vi "Create Accounts Fixture.vi"(8 "error in":errorcluster, 11 "Fixture Name":string) -> (0 "error out":errorcluster, 3 "Accounts File Path":path)   [LabVIEW 2026]
doc: "Test support for the ATM Caraya tests. Writes a fresh accounts file with the four records of the exam specification (12345 John Doe 550, 23456 Jennifer Rodriguez 1000, 34567 Bryan Smith 750, 45678 Julie Ramirez 900) to Tests\\results\\<Fixture Name>.txt and returns its path. The results folder is located relative to this VI (one folder up from Support) and created when missing, so the tests run from any checkout location. An existing fixture file is replaced, so every test starts from the same state. Give every test case its own Fixture Name: Caraya runs the cases of one test VI in parallel."
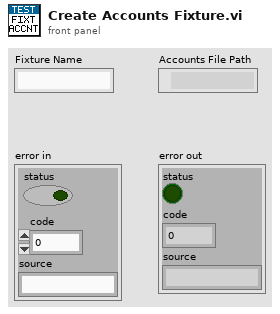
[diagram p1: front panel]
types:
  T1 = enum16{"open", "replace", "create", "open or create", "replace or create", "replace or create with confirmation"}
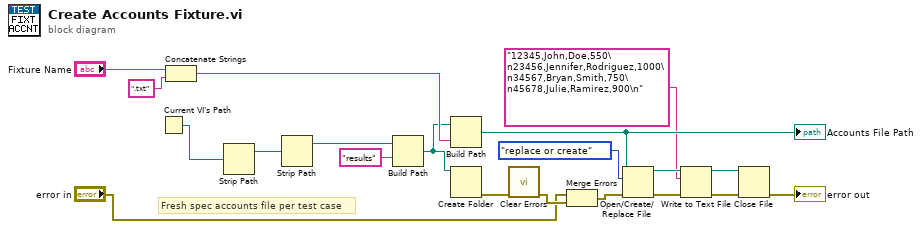
[diagram p0: block diagram]
diagram:
  # "Fresh spec accounts file per test case"
  n1 = Current VI's Path() -> (path=w9:path)
  n2 = Concatenate Strings("Fixture Name", ".txt" ("File Extension")) -> (w16:string)
  n3 = Strip Path(path=w9) -> (stripped path=w10:path)  [unwired: 1 out]
  n4 = Strip Path(path=w10) -> (stripped path=w11:path)  [unwired: 1 out]
  n5 = Build Path(base path=w11, name or relative path="results" ("Results Folder Name")) -> (appended path=w12:path)
  n6 = Build Path(base path=w12, name or relative path=w16) -> (appended path=w7:path)
  "Accounts File Path" <- w7
  n7 = Create Folder(path (use dialog)=w12) -> (error out=w13:errorcluster)  [unwired: 2 in, 2 out]
  n8 = call <vilib>:"Clear Errors.vi"("error in (no error)"=w13) -> ("error out"=w14:errorcluster)  [unwired: 5 in, 1 out]
  n9 = Merge Errors("error in", w14) -> (w15:errorcluster)
  n10 = Open/Create/Replace File(file path (use dialog)=w7, error in=w15, operation (0:open)=T1."replace or create" ("Replace Or Create")) -> (refnum out=w18:refnum<file>, error out=w17:errorcluster)  [unwired: 3 in, 1 out]
  n11 = Write to Text File(file (use dialog)=w18, text="12345,John,Doe,550\n23456,Jennifer,Rodriguez,1000\n34567,Bryan,Smith,750\n45678,Julie,Ramirez,900\n" ("Specification Accounts"), error in=w17) -> (refnum out=w20:refnum<file>, error out=w19:errorcluster)  [unwired: 1 in, 1 out]
  n12 = Close File(refnum=w20, error in=w19) -> (error out=→"error out":errorcluster)  [unwired: 1 out]
